vi "Set PWM Dutty Cycle.Hardware.vi"(8 "error in (no error)":errorcluster, 9 "PWM Timing":cluster{"PWM Range":u32, "PWM Data":u32}, 10 "Duty Cycle (0-1)":dbl=0.5, 11 "RPi PWM Pin in":T1) -> (0 "error out":errorcluster, 3 "RPi PWM Pin out":T1=enum."GPIO2_I2C1_SDA_Pin3")   [LabVIEW 2020, in "wiringPi.lvlib"]
doc: "<b>_______________________________________________________________</b>\n** Author: Juan José Villacorta\n** LabVIEW wrapper for C library <b> wiringPi </b>,\n** https://github.com/WiringPi/WiringPi\n<b>_______________________________________________________________</b>\n\nConfigure a PWM dutty-cycle. Set 0 to stop PWM"
uses:
  wiringPi.lvlib
  Type Defs/GPIO Pins.ctl
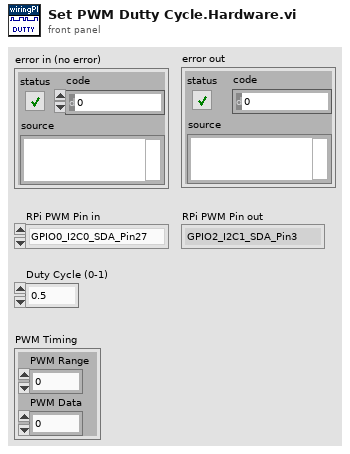
[diagram p1: front panel]
types:
  T1 = typedef "wiringPi.lvlib/GPIO Pins.ctl" = enum32{"GPIO0_I2C0_SDA_Pin27", "GPIO1_I2C0_SDA1_Pin28", "GPIO2_I2C1_SDA_Pin3", "GPIO3_I2C1_SCL_Pin5", "GPIO4_GPCLK0_Pin7", "GPIO5_GPCLK1_Pin29", "GPIO6_GPCLK2_Pin31", "GPIO7_SPI_CE1_N_Pin26", "GPIO8_SPI_CE0_N_Pin24", "GPIO9_SPI0_MISO_Pin21", "GPIO10_SPI0_MOSI_Pin19", "GPIO11_SPI0_CLK_Pin23", "GPIO12_PWM0_Pin32", "GPIO13_PWM1_Pin33", "GPIO14_TXD0_Pin8", "GPIO15_RXD0_Pin10", "GPIO16_Pin36", "GPIO17_Pin11", "GPIO18_PWM0_Pin12", "GPIO19_PWM1_Pin35", "GPIO20_GPCLK0_Pin38", "GPIO21_GPCLK1_Pin40", "GPIO22_Pin15", "GPIO23_Pin16", "GPIO24_Pin18", "GPIO25_Pin22", "GPIO26_Pin37", "GPIO27_Pin13"}
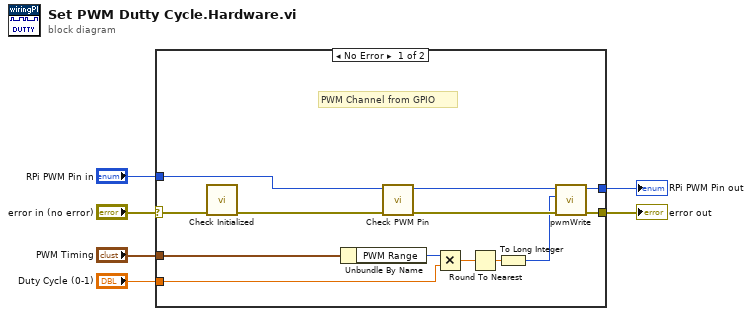
[diagram p0: block diagram]
diagram:
  n1 = case shown="No Error" "error in (no error)" {
    selector: "error in (no error)" -> [w8 w21]
    tunnel: [w13 w21] -> w5
    tunnel: "RPi PWM Pin in" -> [w9 w20]
    tunnel: "PWM Timing" -> [w19 _]
    tunnel: "Duty Cycle (0-1)" -> [w17 _]
    tunnel: [w11 w20] -> w1
    frame No Error {
      # "PWM Channel from GPIO"
      n2 = call "Check Initialized.vi"("error in (no error)"=w8) -> ("error out"=w7:errorcluster)  [unwired: 10 in]
      n3 = Unbundle By Name(w19) -> ("PWM Range"=w18:u32)
      n4 = call "Check PWM Pin.vi"("error in (no error)"=w7, "RPi PWM Pin in"=w9) -> ("error out"=w14:errorcluster, "RPi PWM Pin out"=w10:T1)  [unwired: 8 in]
      n5 = Multiply(x=w18, y=w17) -> (x*y=w15:dbl)
      n6 = Round To Nearest(number=w15) -> (nearest integer value=w16:dbl)
      n7 = To Long Integer(number=w16) -> (32bit integer=w12:i32)
      n8 = call "pwmWrite.vi"("error in (no error)"=w14, "Value"=w12, "RPi Pin"=w10) -> ("error out"=w13:errorcluster, "RPi Pin out"=w11:T1)  [unwired: 7 in]
    }
    frame Error {
    }
  }
  "error out" <- w5
  "RPi PWM Pin out" <- w1
